vi "Stream CreateFlags.vi"(8 "error in (no error)":errorcluster, 11 "StreamFlags":T1) -> (0 "error out":errorcluster, 3 "Stream out":refnum<class "Stream.lvclass">)   [LabVIEW 2020, in "OpenLvVision_OpenCv.lvlib" / "Cuda.lvlib" / "Stream.lvclass"]
doc: "Object by Reference!\nCreates and initializes a new CUDA Stream. \nA stream represents a dedicated, asynchronous execution queue."
uses:
  Stream.lvclass
  C:/Users/lukas/Downloads/OpenLvVision_OpenCv/SourceCode/LabView/OpenLvVision_OpenCv/_LvHelpers/EdvrObject/EdvrObject.lvclass
  TypeDef/Strem Flags.ctl
  _LvHelpers/EdvrObject/TypeDef/Edvr.ctl
  _LvHelpers/EdvrObject/EdvrObject.lvclass/EdvrObject.ctl
  _LvHelpers/EdvrObject/EdvrObject.lvclass
  OpenLvVision_OpenCv.lvlib
  <vilib>/Utility/error.llb/Error Cluster From Error Code.vi
  <vilib>/ErrorRing/Error Ring.xnode
  Dlls/OlvOpenCvWrapper.dll
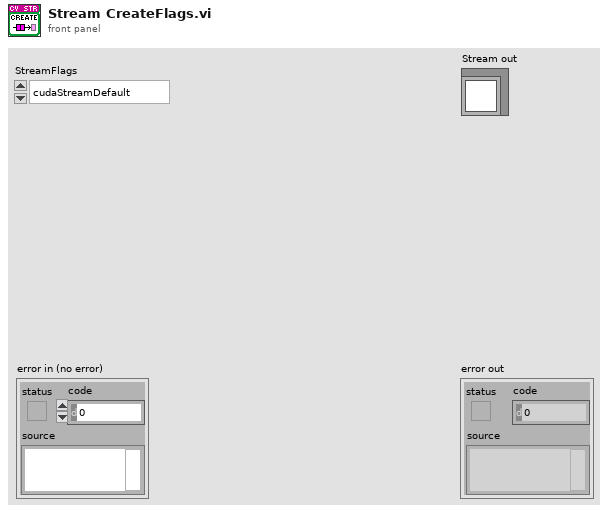
[diagram p1: front panel]
types:
  T1 = typedef "OpenLvVision_OpenCv.lvlib/Strem Flags.ctl" = enum16{"cudaStreamDefault", "cudaStreamNonBlocking"}
  T2 = typedef "OpenLvVision_OpenCv.lvlib/EdvrObject.lvclass/Edvr.ctl" = refnum<data-value>
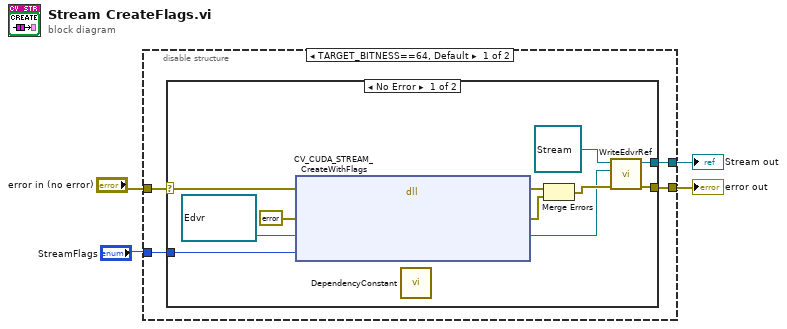
[diagram p0: block diagram]
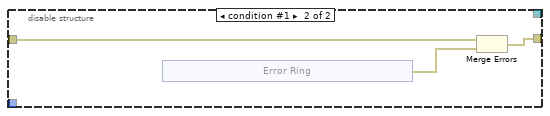
[diagram p3: hidden frame]
diagram:
  n1 = disable-structure shown="TARGET_BITNESS==64, Default" {
    disable-tunnel: "error in (no error)" -> [w8 w22]
    disable-tunnel: [w7 _] -> w4
    disable-tunnel: [w6 w23] -> w3
    disable-tunnel: "StreamFlags" -> [w5 _]
    frame condition #0 (active) {
      n2 = case shown="No Error" w8 {
        selector: w8 -> [w13 w20]
        tunnel: [w19 w20] -> w6
        tunnel: [w18 _] -> w7
        tunnel: w5 -> [w9 _]
        frame No Error {
          n3 = dll-call lib="C:/Users/lukas/Downloads/OpenLvVision_OpenCv/SourceCode/LabView/OpenLvVision_OpenCv/Dlls/OlvOpenCvWrapper.dll" fn="CV_CUDA_STREAM_CreateWithFlags"(error in=w13, "Error"=errorcluster {"status"=FALSE, "code"=0, "source"=""} ("error out"), "edvrRef"=T2 refnum ("Edvr"), "cudaFlags"=w9) -> (error out=w16:errorcluster, "Error"=w10:errorcluster, "edvrRef"=w12:T2)  [unwired: 4 in, 1 out]
          n4 = call "DependencyConstant.vi"() -> ()  [unwired: 12 in]
          n5 = Merge Errors(w16, w10) -> (w14:errorcluster)
          n6 = call "WriteEdvrRef.vi"("error in (no error)"=w14, "Edvr"=w12, "EdvrObject in"=refnum<class "Stream.lvclass"> refnum ("OpenLvVision_OpenCv.lvlib:Cuda.lvlib:Stream")) -> ("error out"=w19:errorcluster, "EdvrObject out"=w18:refnum<class "Stream.lvclass">)  [unwired: 7 in]
        }
        frame Error {
        }
      }
    }
    frame condition #1 {
      n7 = xnode "Error Ring"() -> ("error out"=w21:errorcluster)
      n8 = Merge Errors(w22, w21) -> (w23:errorcluster)
    }
  }
  "error out" <- w3
  "Stream out" <- w4
